vi "BB to Refnum.vi"(3 "BB U64":u64) -> (5 "BB Refnum":T1 {"refnum" format="%.0x"})   [LabVIEW 2021, in "Iceoryx.lvlib"]
uses:
  Iceoryx.lvlib
  Typedef/BB Refnum.ctl
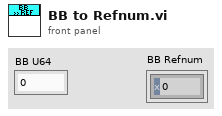
[diagram p1: front panel]
types:
  T1 = typedef "Iceoryx.lvlib/BB Refnum.ctl" = cluster{"refnum":u64, "BB":enum8{"bb"}}
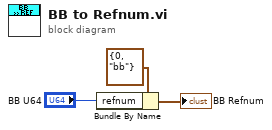
[diagram p0: block diagram]
diagram:
  n1 = Bundle By Name(cluster=T1 {"refnum"=0, "BB"=enum."bb"} ("BB Refnum"), "refnum"="BB U64") -> (→"BB Refnum":T1)
